vi "Main.vi"() -> ()   [LabVIEW 2026]
uses:
  <vilib>/Instr/_visa.llb/VISA Configure Serial Port (Instr).vi
panel:
  out "Estado de Conexión":string
  in  "RESET SLAVE":bool
  out "maquina":T1(ring)
  out "SR MODO":enum16{"AUTOMATICO", "MANUAL"}(ring)=enum."MANUAL"
  out "Boton Reset":string
  out "Errores CRC":dbl
  out "Tramas OK":dbl
  out "Estados de la Planta":string
  out "SALIDA PWM":dbl(graph)
  in  "MODO":bool=TRUE
  in  "RESET":bool
  in  "EMERGENCIA":bool
  in  "PWM":dbl=10.0 min=0.0 max=100.0
  out "SP Vs ALTURA":cluster{dbl, dbl}(graph)
  out "PING PONG":dbl(slide) scale=0.0..50.0
  out "PID":T2(ring)
  out "error out":errorcluster
  out "Enum":enum16{"DESCONECTADO", "CONECTADO"}(ring)
  out "ESTADO  SYS":enum16{"DETENIDO", "EJECUTANDO", "ERROR"}(ring)
  in  "PARADA":bool
  in  "INICIO":bool
  out "PID":string
  in  "SP":dbl=25.0 min=0.0 max=100.0
  in  "KD":dbl=0.07 min=0.0 max=65535.0
  in  "KI":dbl=0.14 min=0.0 max=65535.0
  in  "KP":dbl=3.9 min=0.0 max=65535.0
  in  "PID":bool
  out "PWM (%)":dbl format="%.2g"
  out "ERROR (CM)":dbl format="%.2g"
  out "ALTURA (CM)":dbl format="%.2g"
  out "SP (CM)":dbl format="%.2f"
  out "array":string[][](array[string])
  out "Procesar":string
  in  "Stop Simulation":bool
  in  "Numeric":u32=115200
  in  "VISA resource name":refnum<visa-resource-name>="COM12"
  out "Iteracion":i32
  # "Sistema Levitador Neumático"
  # "Planta"
  # "Grafico en Tiempo Real"
  # "COMUNICACIÓN"
  # "ESTADO DEL SISTEMA"
  # "Estado :"
  # "Puerto :"
  # "Comunicación :"
  # "Baud :"
  # "Estado PID :"
  # "CONFIGURACIÓN PID"
  # "VARIABLES EN TIEMPO REAL"
  # "KP :"
  # "KI :"
  # "KD :"
  # "AUTO"
  # "MANUAL"
  # "SP :"
  # "PWM :"
  # "Mensaje a Procesar :"
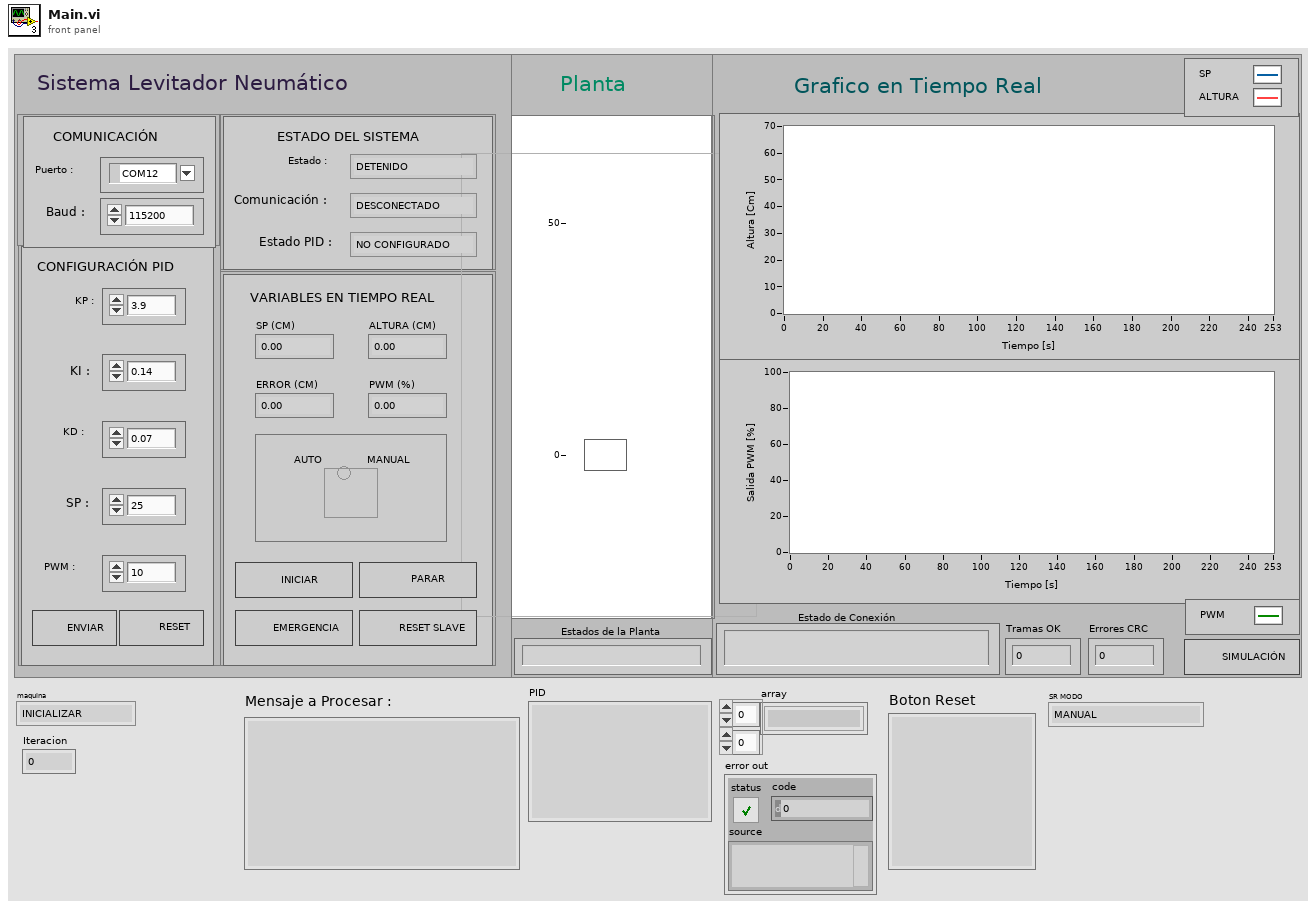
[diagram p1: front panel]
types:
  T1 = enum16{"INICIALIZAR", "ESPERA", "ENVIAR_MODO", "ENVIAR_SP", "ENVIAR_PID", "RECIBIR", "PROCESAR", "ENVIAR_RESET", "ENVIAR_RUN", "ENVIAR_STOP", "ENVIAR_EMERGENCIA_ON", "ENVIAR_EMERGENCIA_OFF", "SLAVE", "ERROR", "CERRAR"}
  T2 = enum16{"NO CONFIGURADO", "CONFIGURADO", "AUTOMATICO"}
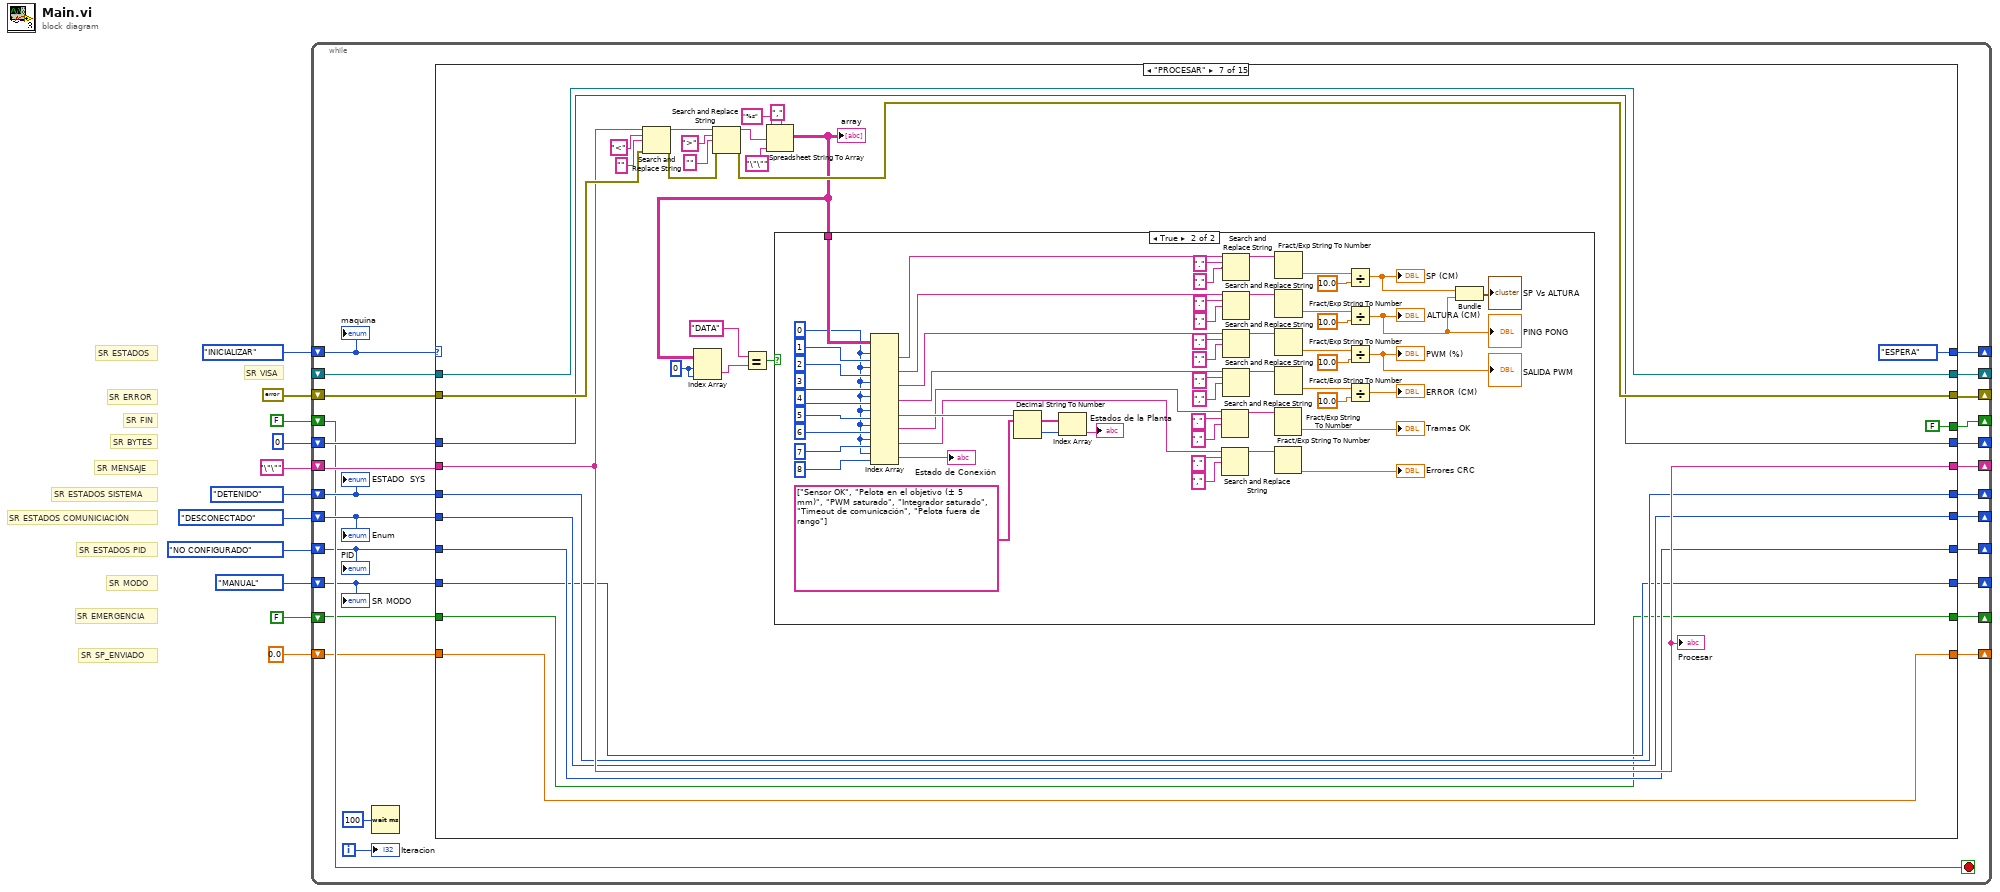
[diagram p0: block diagram]
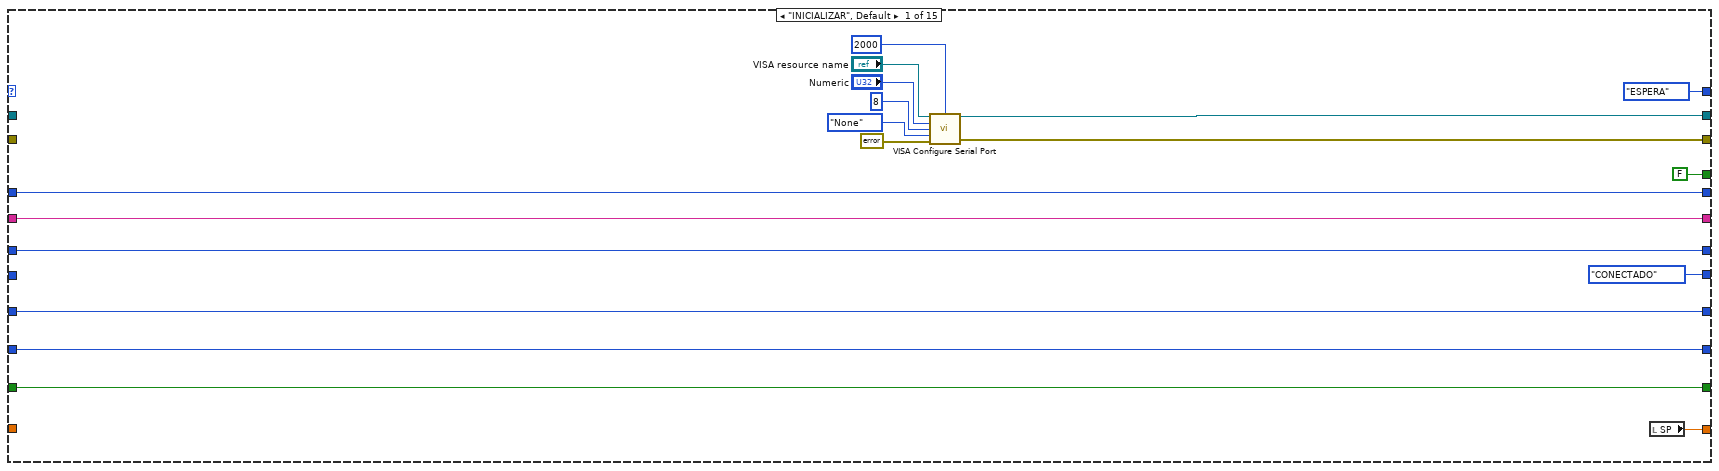
[diagram p2: hidden frame]
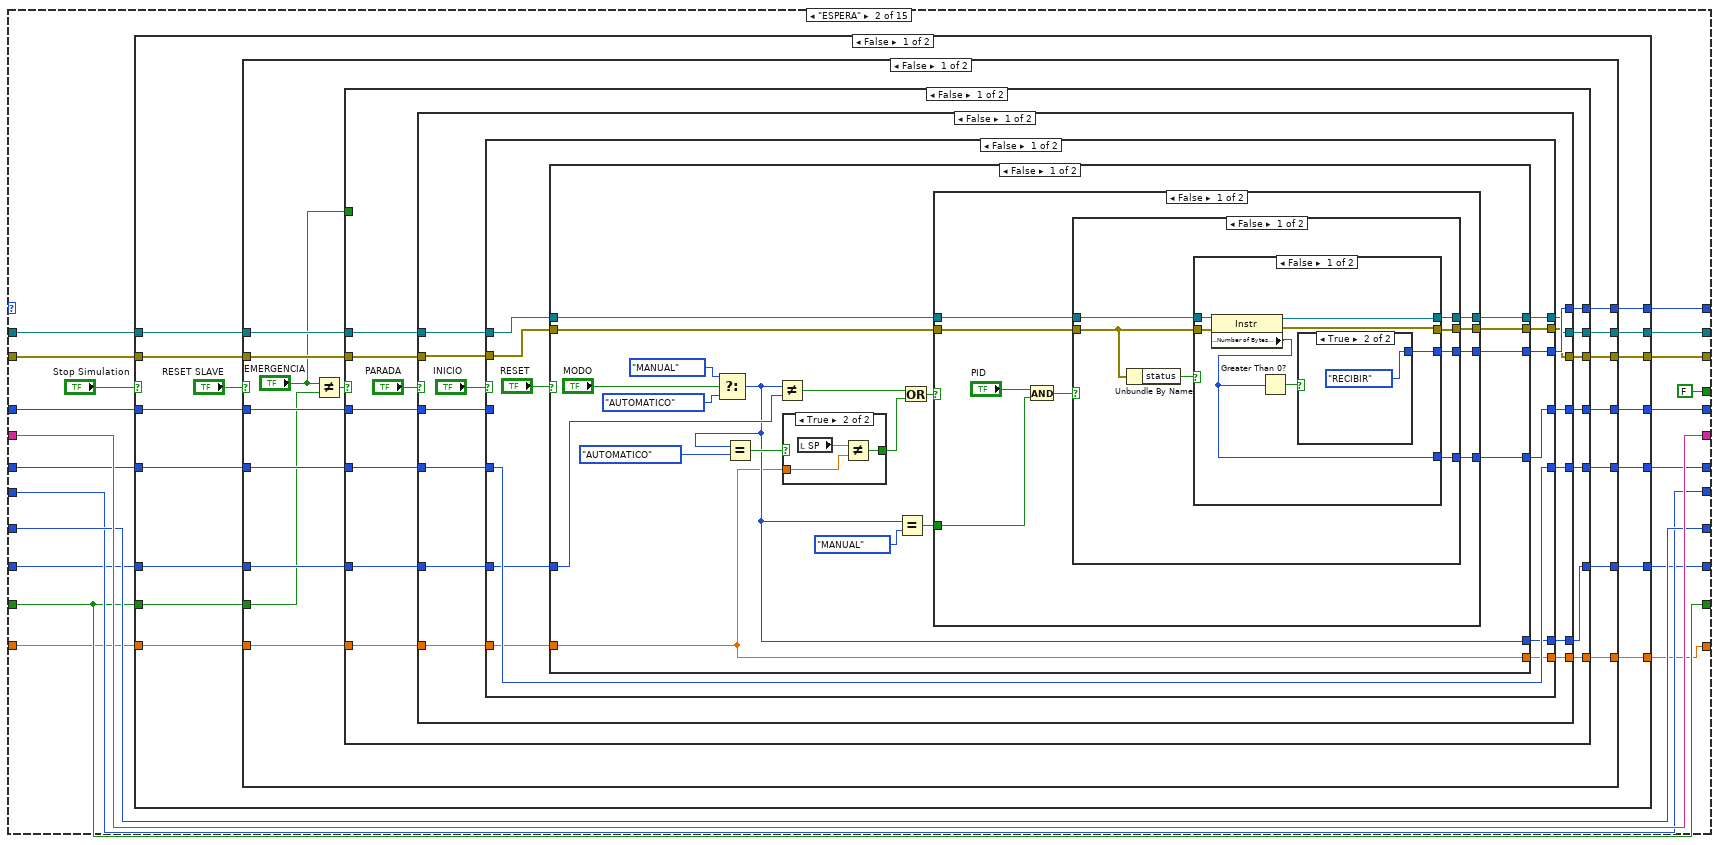
[diagram p3: hidden frame]
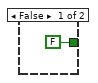
[diagram p4: hidden frame]
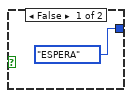
[diagram p5: hidden frame]
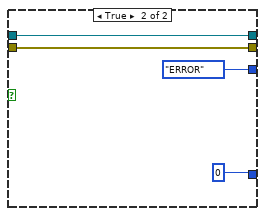
[diagram p6: hidden frame]
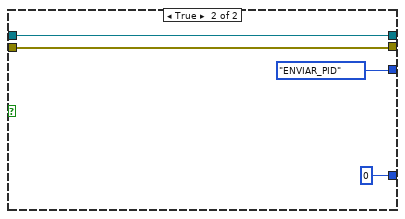
[diagram p7: hidden frame]
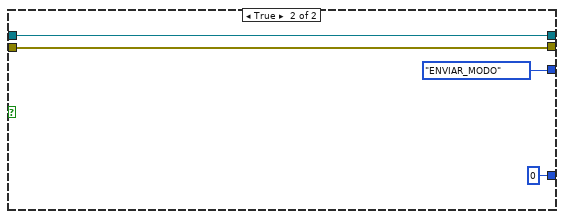
[diagram p8: hidden frame]
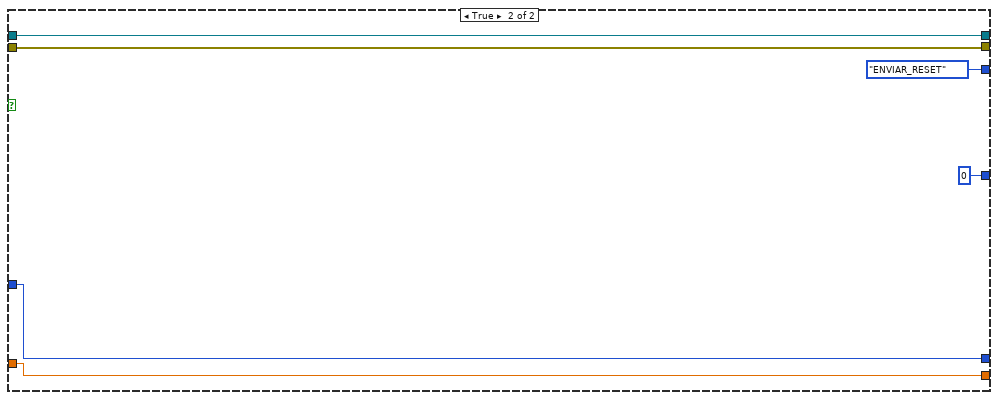
[diagram p9: hidden frame]
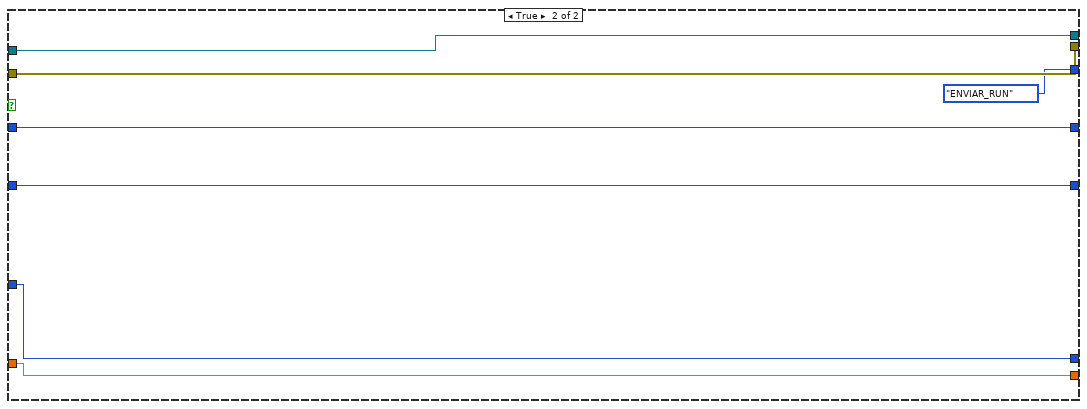
[diagram p10: hidden frame]
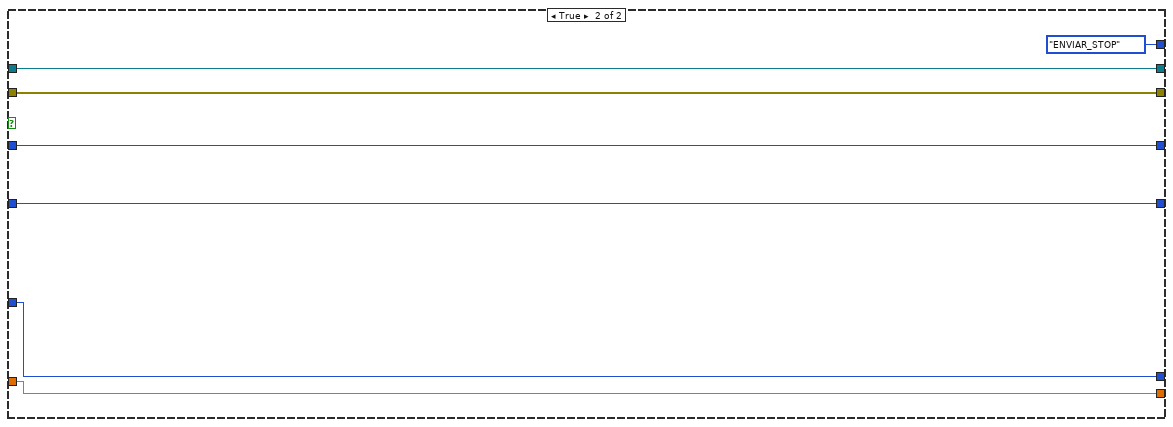
[diagram p11: hidden frame]
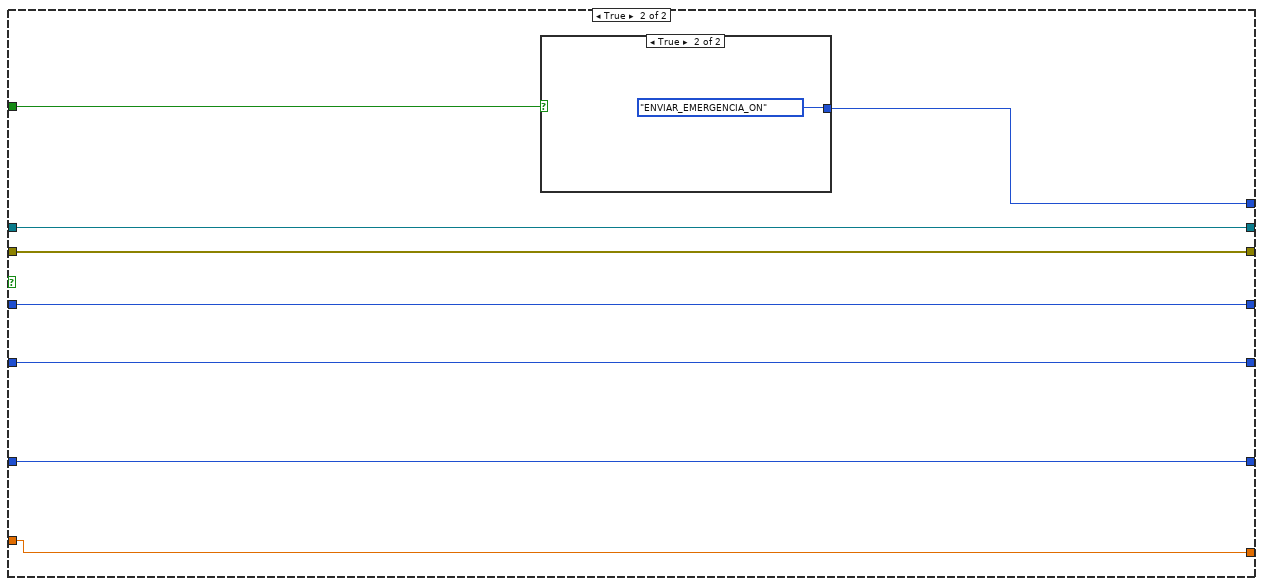
[diagram p12: hidden frame]
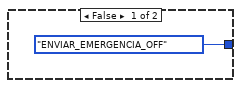
[diagram p13: hidden frame]
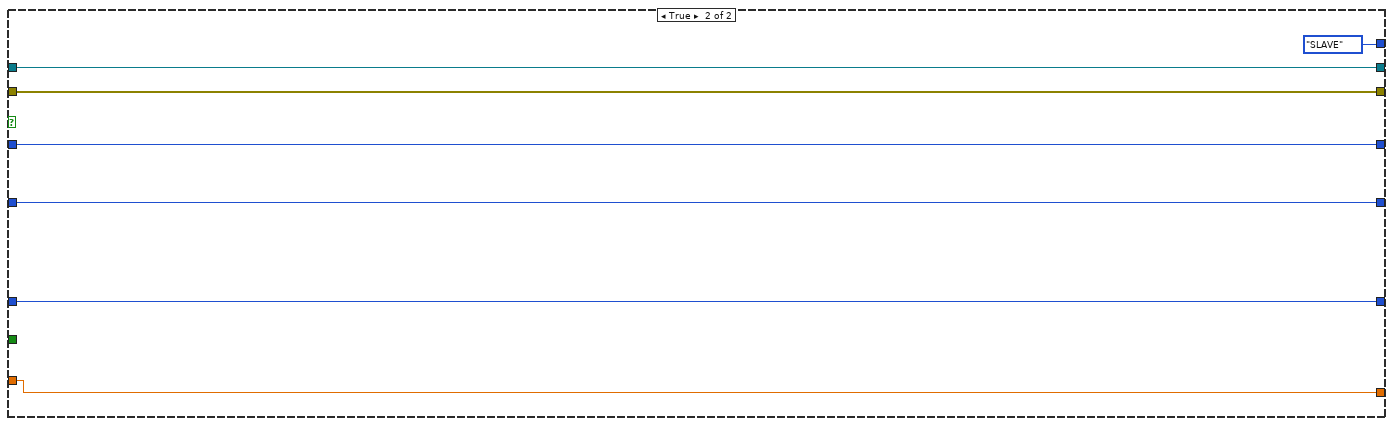
[diagram p14: hidden frame]
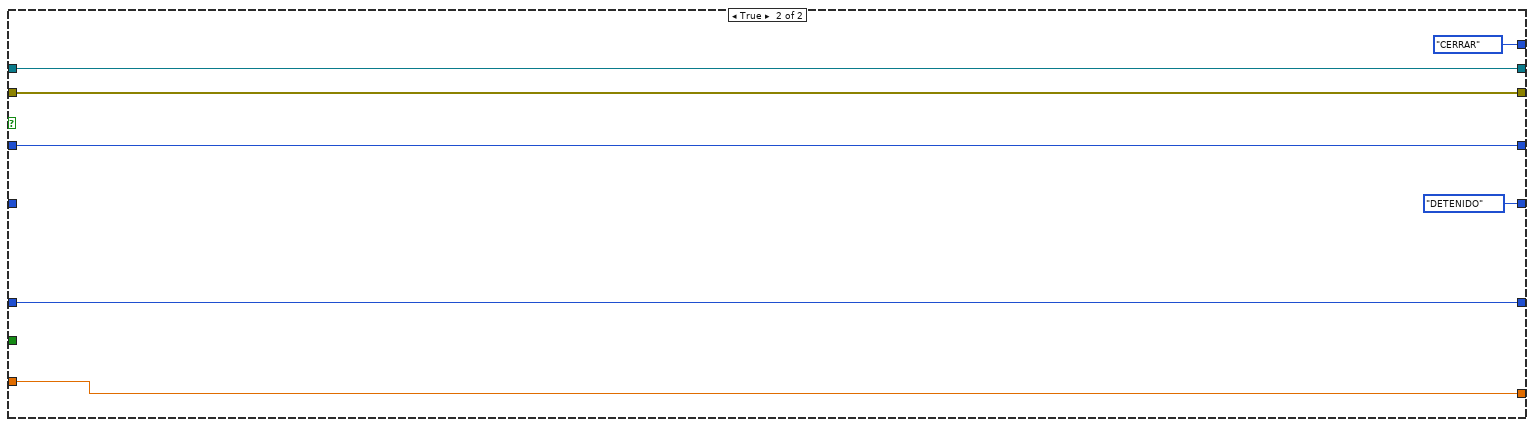
[diagram p15: hidden frame]
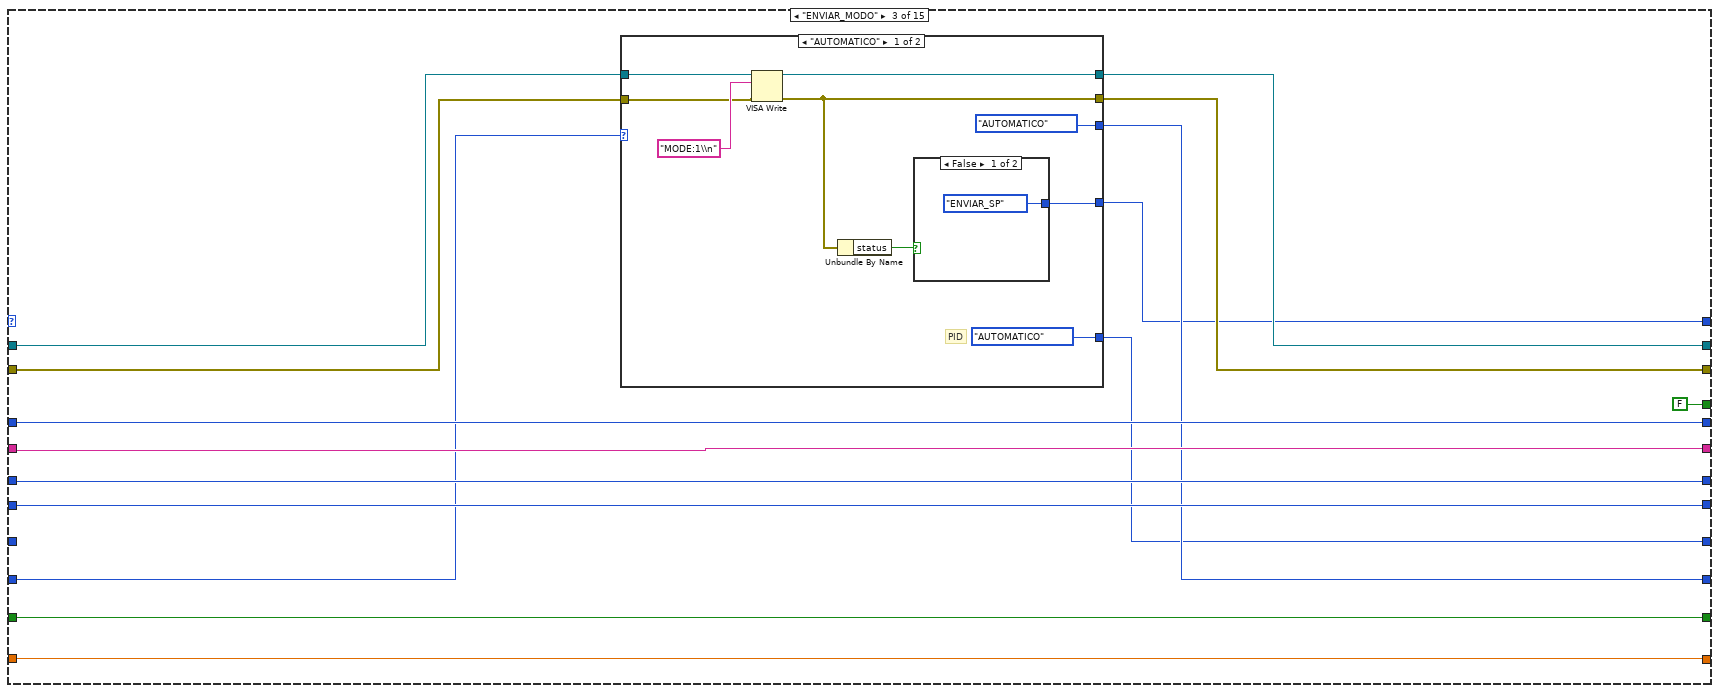
[diagram p16: hidden frame]
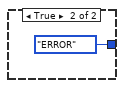
[diagram p17: hidden frame]
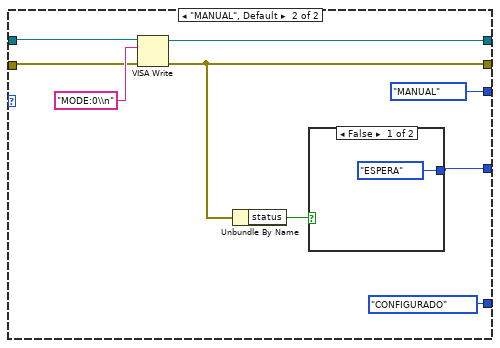
[diagram p18: hidden frame]
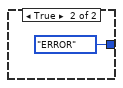
[diagram p19: hidden frame]
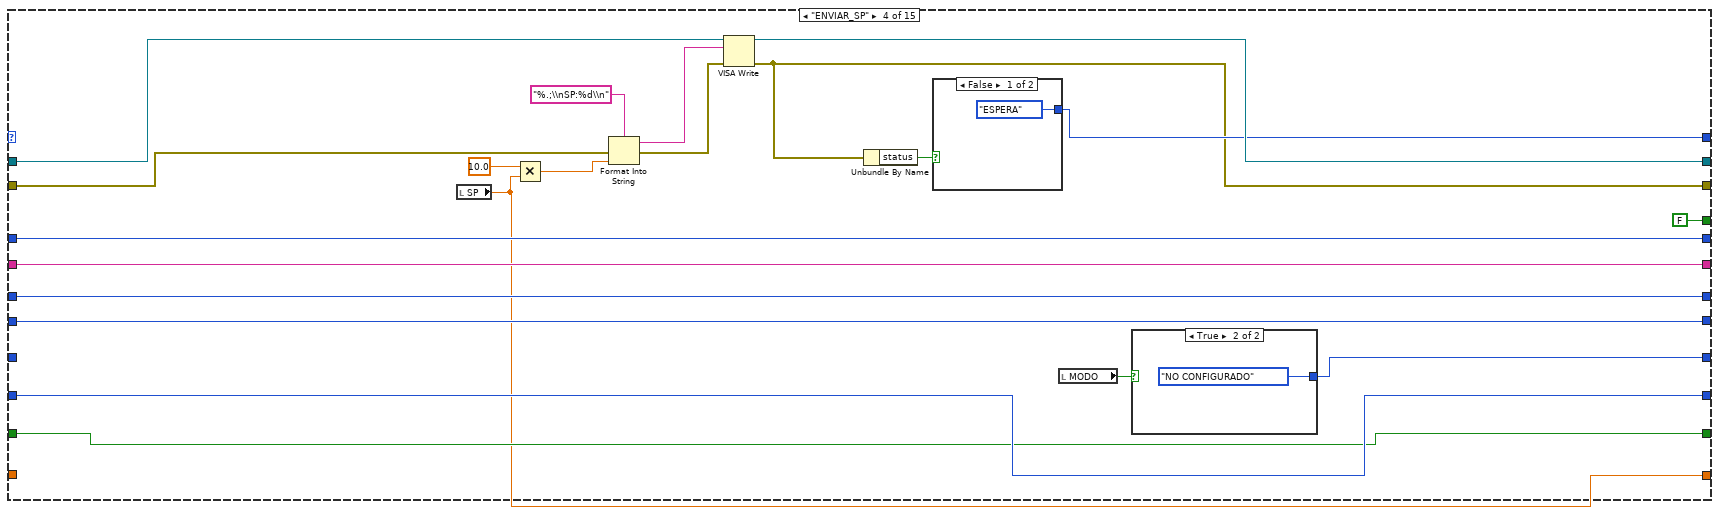
[diagram p20: hidden frame]
diagram:
  # "SR SP_ENVIADO"
  # "SR EMERGENCIA"
  # "SR MODO"
  # "SR ESTADOS PID"
  # "SR ESTADOS COMUNICIACIÓN"
  # "SR ESTADOS SISTEMA"
  # "SR MENSAJE"
  # "SR BYTES"
  # "SR FIN"
  # "SR ERROR"
  # "SR ESTADOS"
  # "SR VISA"
  n1 = while {
    shift-right: [w35] -> _
    shift-left: _ -> [w33]
    shift-right: [w34] -> _
    shift-left: errorcluster {"status"=FALSE, "code"=0, "source"=""} ("error out") -> [w32]
    shift-right: [w31] -> _
    shift-left: FALSE -> [w22]
    shift-right: [w30] -> _
    shift-left: u32 0 ("Bytes at Port") -> [w29]
    shift-right: [w28] -> _
    shift-left: "\"\"" -> [w27]
    shift-right: [w23] -> _
    shift-left: enum16{"DETENIDO", "EJECUTANDO", "ERROR"}."DETENIDO" -> [w25]
    shift-right: [w24] -> _
    shift-left: enum16{"DESCONECTADO", "CONECTADO"}."DESCONECTADO" -> [w26]
    shift-right: [w20] -> _
    shift-left: T2."NO CONFIGURADO" -> [w21]
    shift-right: [w18] -> _
    shift-left: T1."INICIALIZAR" -> [w19]
    shift-right: [w16] -> _
    shift-left: enum16{"AUTOMATICO", "MANUAL"}."MANUAL" -> [w17]
    shift-right: [w14] -> _
    shift-left: FALSE -> [w15]
    shift-right: [w12] -> _
    shift-left: 0.0 -> [w13]
    i -> [w37]
    stop <- w22 stop-if-true
    n2 = Wait (ms)(milliseconds to wait=u32 100) -> ()  [unwired: 1 out]
    n3 = case shown="\"PROCESAR\"" w19 {
      tunnel: [T1."ESPERA" w59 w253 w293 w333 w353 T1."ESPERA" w455 w476 w492 w512 w530 T1."CERRAR" T1."CERRAR" w567] -> w18
      tunnel: [w49 w72 w257 w294 w338 w358 w391 w457 w478 w493 w509 w532 w550 w556 w566] -> w35
      tunnel: [w48 w71 w256 w292 w335 w355 w382 w452 w477 w494 w508 w531 w546 w557 w565] -> w34
      tunnel: w33 -> [_ w73 w259 w296 w339 w360 w391 w459 w480 w498 w514 w534 w550 w556 w569]
      tunnel: w32 -> [_ w67 w258 w295 w341 w359 w383 w458 w479 w497 w513 w533 w546 w558 w568]
      tunnel: [FALSE FALSE FALSE FALSE FALSE FALSE FALSE FALSE FALSE FALSE FALSE FALSE FALSE TRUE FALSE] -> w31
      tunnel: [w46 w70 w262 w304 w343 w357 w378 w448 w473 w495 w510 w527 w548 w562 w570] -> w30
      tunnel: w29 -> [w46 w69 w262 w304 w343 w357 w378 w448 w473 w495 w510 w527 w548 w562 w570]
      tunnel: [w45 w68 w263 w305 w342 w356 w376 w454 w474 w496 w507 w526 w547 w561 w571] -> w28
      tunnel: w27 -> [w45 w68 w263 w305 w342 _ w376 w454 w474 w496 w507 w526 w547 w561 w571]
      tunnel: w25 -> [w44 w65 w261 w307 w332 w352 w370 w453 _ _ _ w523 w545 _ w572]
      tunnel: w26 -> [_ w62 w260 w303 w316 w350 w368 w451 w470 w488 w506 w524 w543 _ w573]
      tunnel: [enum16{"DESCONECTADO", "CONECTADO"}."CONECTADO" w62 w260 w303 w316 w350 w368 w451 w470 w488 w506 w524 w543 enum16{"DESCONECTADO", "CONECTADO"}."DESCONECTADO" w573] -> w24
      tunnel: [w44 w66 w261 w307 w332 w352 w370 w453 enum16{"DETENIDO", "EJECUTANDO", "ERROR"}."EJECUTANDO" enum16{"DETENIDO", "EJECUTANDO", "ERROR"}."DETENIDO" enum16{"DETENIDO", "EJECUTANDO", "ERROR"}."DETENIDO" w523 w545 enum16{"DETENIDO", "EJECUTANDO", "ERROR"}."DETENIDO" w572] -> w23
      tunnel: w21 -> [w43 w63 _ _ _ w351 w369 _ w471 w489 w511 w528 w544 w555 w574]
      tunnel: [w43 w63 w252 w291 T2."CONFIGURADO" w351 w369 T2."NO CONFIGURADO" w471 w489 w511 w528 w544 w555 w574] -> w20
      tunnel: w17 -> [w41 w61 w254 w289 w314 w349 w367 w449 w469 w487 w505 w525 w542 w554 w575]
      tunnel: [w41 w60 w255 w289 w314 w349 w367 w449 w469 w487 w505 w525 w542 w554 w575] -> w16
      tunnel: w15 -> [w40 w58 w251 w288 w313 w348 w366 w447 w468 w486 _ _ w541 w553 _]
      tunnel: [w40 w58 w251 w288 w313 w348 w366 w447 w468 w486 TRUE FALSE w541 w553 FALSE] -> w14
      tunnel: w13 -> [_ w57 w250 _ w312 w347 w365 w446 w467 w485 w503 w521 w540 w552 w576]
      tunnel: [w39 w56 w250 w287 w312 w347 w365 w446 w467 w485 w503 w521 w540 w552 w576] -> w12
      frame "INICIALIZAR", Default {
        n4 = call-poly "VISA Configure Serial Port"("VISA resource name"="VISA resource name", "timeout (10sec)"=u32 2000, "baud rate (9600)"="Numeric", "data bits (8)"=u16 8, "parity (0:none)"=enum16{"None", "Odd", "Even", "Mark", "Space"}."None", "error in (no error)"=errorcluster {"status"=FALSE, "code"=0, "source"=""}) -> ("VISA resource name out"=w49:refnum<visa-resource-name>, "error out"=w48:errorcluster)  [unwired: 8 in]
        n5 = local read "SP"() -> (w39:dbl)
      }
      frame "ESPERA" {
        n6 = case shown="False" "Stop Simulation" {
          tunnel: [w89 T1."CERRAR"] -> w59
          tunnel: w73 -> [w88 w247]
          tunnel: [w87 w247] -> w72
          tunnel: [w86 w246] -> w71
          tunnel: [w85 w249] -> w70
          tunnel: w69 -> [w84 w249]
          tunnel: w67 -> [w83 w246]
          tunnel: [w82 enum16{"DETENIDO", "EJECUTANDO", "ERROR"}."DETENIDO"] -> w66
          tunnel: w65 -> [w81 _]
          tunnel: w61 -> [w80 w245]
          tunnel: [w79 w245] -> w60
          tunnel: w58 -> [w78 _]
          tunnel: w57 -> [w77 w244]
          tunnel: [w76 w244] -> w56
          frame False {
            n7 = case shown="False" "RESET SLAVE" {
              tunnel: [w105 T1."SLAVE"] -> w89
              tunnel: w88 -> [w104 w237]
              tunnel: [w103 w237] -> w87
              tunnel: [w102 w238] -> w86
              tunnel: [w101 w239] -> w85
              tunnel: w84 -> [w100 w239]
              tunnel: w83 -> [w99 w238]
              tunnel: [w98 w240] -> w82
              tunnel: w81 -> [w97 w240]
              tunnel: w80 -> [w96 w241]
              tunnel: [w95 w241] -> w79
              tunnel: w78 -> [w93 _]
              tunnel: w77 -> [w91 w242]
              tunnel: [w90 w242] -> w76
              frame False {
                n8 = Not Equal?(x="EMERGENCIA", y=w93) -> (x != y?=w94:bool)
                n9 = case shown="False" w94 {
                  tunnel: [w119 w228] -> w105
                  tunnel: w104 -> [w111 w231]
                  tunnel: [w118 w231] -> w103
                  tunnel: [w117 w230] -> w102
                  tunnel: [w116 w233] -> w101
                  tunnel: w100 -> [w115 w233]
                  tunnel: w99 -> [w110 w230]
                  tunnel: [w113 w232] -> w98
                  tunnel: w97 -> [w112 w232]
                  tunnel: w96 -> [w109 w229]
                  tunnel: [w108 w229] -> w95
                  tunnel: "EMERGENCIA" -> [_ w227]
                  tunnel: w91 -> [w107 w226]
                  tunnel: [w106 w226] -> w90
                  frame False {
                    n10 = case shown="False" "PARADA" {
                      tunnel: [w133 T1."ENVIAR_STOP"] -> w119
                      tunnel: w111 -> [w132 w225]
                      tunnel: w110 -> [w131 w224]
                      tunnel: [w130 w225] -> w118
                      tunnel: [w129 w224] -> w117
                      tunnel: [w128 w223] -> w116
                      tunnel: w115 -> [w126 w223]
                      tunnel: [w125 w222] -> w113
                      tunnel: w112 -> [w124 w222]
                      tunnel: w109 -> [w123 w221]
                      tunnel: [w122 w221] -> w108
                      tunnel: w107 -> [w121 w220]
                      tunnel: [w120 w220] -> w106
                      frame False {
                        n11 = case shown="False" "INICIO" {
                          tunnel: [w145 T1."ENVIAR_RUN"] -> w133
                          tunnel: w132 -> [w144 w218]
                          tunnel: w131 -> [w143 w217]
                          tunnel: [w142 w218] -> w130
                          tunnel: [w141 w217] -> w129
                          tunnel: [w140 w216] -> w128
                          tunnel: w126 -> [_ w216]
                          tunnel: [w139 w215] -> w125
                          tunnel: w124 -> [w139 w215]
                          tunnel: w123 -> [w137 w214]
                          tunnel: [w136 w214] -> w122
                          tunnel: w121 -> [w135 w213]
                          tunnel: [w134 w213] -> w120
                          frame False {
                            n12 = case shown="False" "RESET" {
                              tunnel: [w164 T1."ENVIAR_RESET"] -> w145
                              tunnel: w144 -> [w163 w211]
                              tunnel: w143 -> [w162 w210]
                              tunnel: [w161 w211] -> w142
                              tunnel: [w160 w210] -> w141
                              tunnel: [w159 u32 0 ("Bytes at Port")] -> w140
                              tunnel: w137 -> [w155 w208]
                              tunnel: [w148 w208] -> w136
                              tunnel: w135 -> [w146 w207]
                              tunnel: [w146 w207] -> w134
                              frame False {
                                n13 = Select(t=enum16{"AUTOMATICO", "MANUAL"}."MANUAL", s="MODO", f=enum16{"AUTOMATICO", "MANUAL"}."AUTOMATICO") -> (s? t:f=w148:enum16{"AUTOMATICO", "MANUAL"})
                                n14 = Equal?(x=w148, y=enum16{"AUTOMATICO", "MANUAL"}."AUTOMATICO") -> (x = y?=w149:bool)
                                n15 = Not Equal?(x=w148, y=w155) -> (x != y?=w151:bool)
                                n16 = case shown="True" w149 {
                                tunnel: [FALSE w167] -> w152
                                tunnel: w146 -> [_ w166]
                                frame False {
                                }
                                frame True {
                                n17 = local read "SP"() -> (w168:dbl)
                                n18 = Not Equal?(x=w168, y=w166) -> (x != y?=w167:bool)
                                }
                                }
                                n19 = Equal?(x=w148, y=enum16{"AUTOMATICO", "MANUAL"}."MANUAL") -> (x = y?=w154:bool)
                                n20 = Or(x=w151, y=w152) -> (x .or. y?=w150:bool)
                                n21 = case shown="False" w150 {
                                tunnel: [w177 T1."ENVIAR_MODO"] -> w164
                                tunnel: w163 -> [w176 w205]
                                tunnel: w162 -> [w175 w204]
                                tunnel: [w174 w205] -> w161
                                tunnel: [w173 w204] -> w160
                                tunnel: [w172 u32 0 ("Bytes at Port")] -> w159
                                tunnel: w154 -> [w171 _]
                                frame False {
                                n22 = And(x="PID", y=w171) -> (x .and. y?=w169:bool)
                                n23 = case shown="False" w169 {
                                tunnel: [w184 T1."ENVIAR_PID"] -> w177
                                tunnel: w176 -> [w183 w200]
                                tunnel: w175 -> [w179 w199]
                                tunnel: [w182 w200] -> w174
                                tunnel: [w181 w199] -> w173
                                tunnel: [w180 u32 0 ("Bytes at Port")] -> w172
                                frame False {
                                n24 = Unbundle By Name(w179) -> ("status"=w178:bool)
                                n25 = case shown="False" w178 {
                                tunnel: [w191 T1."ERROR"] -> w184
                                tunnel: w183 -> [w190 w197]
                                tunnel: w179 -> [w189 w196]
                                tunnel: [w188 w197] -> w182
                                tunnel: [w187 w196] -> w181
                                tunnel: [w185 u32 0 ("Bytes at Port")] -> w180
                                frame False {
                                n26 = property class="Instr"(reference=w190, error in=w189) -> (reference out=w188:refnum<visa-resource-name>, error out=w187:errorcluster, "Serial Settings:Number of Bytes at Serial Port"=w185:u32)
                                n27 = Greater Than 0?(x=w185) -> (x > 0?=w186:bool)
                                n28 = case shown="True" w186 {
                                tunnel: [T1."ESPERA" T1."RECIBIR"] -> w191
                                frame False {
                                }
                                frame True {
                                }
                                }
                                }
                                frame True {
                                }
                                }
                                }
                                frame True {
                                }
                                }
                                }
                                frame True {
                                }
                                }
                              }
                              frame True {
                              }
                            }
                          }
                          frame True {
                          }
                        }
                      }
                      frame True {
                      }
                    }
                  }
                  frame True {
                    n29 = case shown="True" w227 {
                      tunnel: [T1."ENVIAR_EMERGENCIA_OFF" T1."ENVIAR_EMERGENCIA_ON"] -> w228
                      frame False {
                      }
                      frame True {
                      }
                    }
                  }
                }
              }
              frame True {
              }
            }
          }
          frame True {
          }
        }
      }
      frame "ENVIAR_MODO" {
        n30 = case shown="\"AUTOMATICO\"" w254 {
          tunnel: w259 -> [w271 w283]
          tunnel: w258 -> [w270 w282]
          tunnel: [w269 w280] -> w257
          tunnel: [w268 w281] -> w256
          tunnel: [enum16{"AUTOMATICO", "MANUAL"}."AUTOMATICO" enum16{"AUTOMATICO", "MANUAL"}."MANUAL"] -> w255
          tunnel: [w266 w277] -> w253
          tunnel: [T2."AUTOMATICO" T2."CONFIGURADO"] -> w252
          frame "AUTOMATICO" {
            # "PID"
            n31 = VISA Write(VISA resource name=w271, write buffer="MODE:1\\n", error in (no error)=w270) -> (VISA resource name out=w269:refnum<visa-resource-name>, error out=w268:errorcluster)  [unwired: 1 out]
            n32 = Unbundle By Name(w268) -> ("status"=w272:bool)
            n33 = case shown="False" w272 {
              tunnel: [T1."ENVIAR_SP" T1."ERROR"] -> w266
              frame False {
              }
              frame True {
              }
            }
          }
          frame "MANUAL", Default {
            n34 = VISA Write(VISA resource name=w283, write buffer="MODE:0\\n", error in (no error)=w282) -> (VISA resource name out=w280:refnum<visa-resource-name>, error out=w281:errorcluster)  [unwired: 1 out]
            n35 = Unbundle By Name(w281) -> ("status"=w279:bool)
            n36 = case shown="False" w279 {
              tunnel: [T1."ESPERA" T1."ERROR"] -> w277
              frame False {
              }
              frame True {
              }
            }
          }
        }
      }
      frame "ENVIAR_SP" {
        n37 = local read "SP"() -> (w287:dbl)
        n38 = Multiply(x=10.0, y=w287) -> (x*y=w300:dbl)
        n39 = Format Into String(format string="%.;\\nSP:%d\\n", error in=w295, w300) -> (resulting string=w302:string, error out=w301:errorcluster)  [unwired: 1 in]
        n40 = VISA Write(VISA resource name=w296, write buffer=w302, error in (no error)=w301) -> (VISA resource name out=w294:refnum<visa-resource-name>, error out=w292:errorcluster)  [unwired: 1 out]
        n41 = Unbundle By Name(w292) -> ("status"=w299:bool)
        n42 = case shown="False" w299 {
          tunnel: [T1."ESPERA" T1."ERROR"] -> w293
          frame False {
          }
          frame True {
          }
        }
        n43 = local read "MODO"() -> (w290:bool)
        n44 = case shown="True" w290 {
          tunnel: [T2."AUTOMATICO" T2."NO CONFIGURADO"] -> w291
          frame False {
          }
          frame True {
          }
        }
      }
      frame "ENVIAR_PID" {
        n45 = Multiply(x=100.0, y="KP") -> (x*y=w323:dbl)
        n46 = Multiply(x=100.0, y="KI") -> (x*y=w327:dbl)
        n47 = Multiply(x=100.0, y="KD") -> (x*y=w331:dbl)
        n48 = Multiply(x=10.0, y="SP") -> (x*y=w320:dbl)
        n49 = Multiply(x=10.0, y="PWM") -> (x*y=w317:dbl)
        n50 = Format Into String(format string="%.;\\nKP:%d\\nKI:%d\\nKD:%d\\nSP:%d\\nPWM:%d\\n", error in=w341, w323, w327, w331, w320, w317) -> (resulting string=w340:string, error out=w336:errorcluster)  [unwired: 1 in]
        "PID" <- w340
        n51 = VISA Write(VISA resource name=w339, write buffer=w340, error in (no error)=w336) -> (VISA resource name out=w338:refnum<visa-resource-name>, error out=w335:errorcluster)  [unwired: 1 out]
        n52 = Unbundle By Name(w335) -> ("status"=w334:bool)
        n53 = case shown="False" w334 {
          tunnel: [T1."ESPERA" T1."ERROR"] -> w333
          frame False {
          }
          frame True {
          }
        }
      }
      frame "RECIBIR" {
        n54 = VISA Read(VISA resource name=w360, byte count=w357, error in (no error)=w359) -> (VISA resource name out=w358:refnum<visa-resource-name>, read buffer=w356:string, error out=w355:errorcluster)  [unwired: 1 out]
        n55 = Unbundle By Name(w355) -> ("status"=w354:bool)
        n56 = case shown="False" w354 {
          tunnel: [T1."PROCESAR" T1."ERROR"] -> w353
          frame False {
          }
          frame True {
          }
        }
      }
      frame "PROCESAR" {
        w375 = 0 ("index (row)")
        n57 = Search and Replace String(input string=w376, search string="<", replace string="" ("replace string (\"\")"), error in=w383) -> (result string=w387:string, error out=w386:errorcluster)  [unwired: 4 in, 2 out]
        n58 = Search and Replace String(input string=w387, search string=">", replace string="" ("replace string (\"\")"), error in=w386) -> (result string=w380:string, error out=w382:errorcluster)  [unwired: 4 in, 2 out]
        n59 = Spreadsheet String To Array(delimiter (Tab)=",", format string="%s", spreadsheet string=w380, array type (2D Dbl)="\"\"") -> (array=w371:string[][])
        "array" <- w371
        n60 = Index Array(array=w371, index (row)=w375, index (col)=w375) -> (element=w374:string)
        n61 = Equal?(x="DATA", y=w374) -> (x = y?=w372:bool)
        n62 = case shown="True" w372 {
          tunnel: w371 -> [_ w424]
          frame False {
          }
          frame True {
            w394 = 0 ("index (row)")
            n63 = Index Array(array=w424, index (row) #1=w394, index (col) #1=1 ("index"), index (row) #2=w394, index (col) #2=2 ("index"), index (row) #3=w394, index (col) #3=3 ("index"), index (row) #4=w394, index (col) #4=4 ("index"), index (row) #5=w394, index (col) #5=5 ("disabled index (col)"), index (row) #6=w394, index (col) #6=6 ("disabled index (col)"), index (row) #7=w394, index (col) #7=7 ("disabled index (col)"), index (row) #8=w394, index (col) #8=8 ("disabled index (col)")) -> (element #1=w441:string, element #2=w432:string, element #3=w431:string, element #4=w430:string, element #5=w420:string, element #6=w408:string, element #7=w407:string, element #8=→"Estado de Conexión":string)
            n64 = Decimal String To Number(string=w420) -> (number=w418:i32)  [unwired: 2 in, 1 out]
            n65 = Index Array(array=string[] ["Sensor OK", "Pelota en el objetivo (± 5 mm)", "PWM saturado", "Integrador saturado", "Timeout de comunicación", "Pelota fuera de rango"], index=w418) -> (element=→"Estados de la Planta":string)
            n66 = Search and Replace String(input string=w408, search string=".", replace string="," ("replace string (\"\")")) -> (result string=w410:string)  [unwired: 5 in, 3 out]
            n67 = Search and Replace String(input string=w407, search string=".", replace string="," ("replace string (\"\")")) -> (result string=w409:string)  [unwired: 5 in, 3 out]
            n68 = Search and Replace String(input string=w441, search string=".", replace string="," ("replace string (\"\")")) -> (result string=w439:string)  [unwired: 5 in, 3 out]
            n69 = Search and Replace String(input string=w432, search string=".", replace string="," ("replace string (\"\")")) -> (result string=w428:string)  [unwired: 5 in, 3 out]
            n70 = Search and Replace String(input string=w431, search string=".", replace string="," ("replace string (\"\")")) -> (result string=w427:string)  [unwired: 5 in, 3 out]
            n71 = Search and Replace String(input string=w430, search string=".", replace string="," ("replace string (\"\")")) -> (result string=w426:string)  [unwired: 5 in, 3 out]
            n72 = Fract/Exp String To Number(string=w410) -> (number=→"Tramas OK":dbl)  [unwired: 3 in, 1 out]
            n73 = Fract/Exp String To Number(string=w409) -> (number=→"Errores CRC":dbl)  [unwired: 3 in, 1 out]
            n74 = Fract/Exp String To Number(string=w439) -> (number=w422:dbl)  [unwired: 3 in, 1 out]
            n75 = Fract/Exp String To Number(string=w428) -> (number=w402:dbl)  [unwired: 3 in, 1 out]
            n76 = Fract/Exp String To Number(string=w427) -> (number=w399:dbl)  [unwired: 3 in, 1 out]
            n77 = Fract/Exp String To Number(string=w426) -> (number=w396:dbl)  [unwired: 3 in, 1 out]
            n78 = Divide(x=w422, y=10.0) -> (x/y=w404:dbl)
            "SP (CM)" <- w404
            n79 = Divide(x=w402, y=10.0) -> (x/y=w401:dbl)
            "ALTURA (CM)" <- w401
            "PING PONG" <- w401
            n80 = Divide(x=w399, y=10.0) -> (x/y=→"PWM (%)" →"SALIDA PWM":dbl)
            n81 = Divide(x=w396, y=10.0) -> (x/y=→"ERROR (CM)":dbl)
            n82 = Bundle(w404, w401) -> (→"SP Vs ALTURA":cluster{dbl, dbl})  [unwired: 1 in]
          }
        }
        "Procesar" <- w376
      }
      frame "ENVIAR_RESET" {
        w460 = 0.0 ("input 1")
        n83 = Format Into String(format string="%.;\\nKP:%d\\nKI:%d\\nKD:%d\\nSP:%d\\nPWM:%d\\n", error in=w458, w460, w460, w460, w460, w460) -> (resulting string=w464:string, error out=w462:errorcluster)  [unwired: 1 in]
        "Boton Reset" <- w464
        n84 = VISA Write(VISA resource name=w459, write buffer=w464, error in (no error)=w462) -> (VISA resource name out=w457:refnum<visa-resource-name>, error out=w452:errorcluster)  [unwired: 1 out]
        n85 = Unbundle By Name(w452) -> ("status"=w461:bool)
        n86 = case shown="False" w461 {
          tunnel: [T1."ESPERA" T1."ERROR"] -> w455
          frame False {
          }
          frame True {
          }
        }
      }
      frame "ENVIAR_RUN" {
        n87 = VISA Write(VISA resource name=w480, write buffer="EN:1\\n", error in (no error)=w479) -> (VISA resource name out=w478:refnum<visa-resource-name>, error out=w477:errorcluster)  [unwired: 1 out]
        n88 = Unbundle By Name(w477) -> ("status"=w482:bool)
        n89 = case shown="False" w482 {
          tunnel: [T1."ESPERA" T1."ERROR"] -> w476
          frame False {
          }
          frame True {
          }
        }
      }
      frame "ENVIAR_STOP" {
        n90 = VISA Write(VISA resource name=w498, write buffer="EN:0\\n", error in (no error)=w497) -> (VISA resource name out=w493:refnum<visa-resource-name>, error out=w494:errorcluster)  [unwired: 1 out]
        n91 = Unbundle By Name(w494) -> ("status"=w500:bool)
        n92 = case shown="False" w500 {
          tunnel: [T1."ESPERA" T1."ERROR"] -> w492
          frame False {
          }
          frame True {
          }
        }
      }
      frame "ENVIAR_EMERGENCIA_ON" {
        n93 = VISA Write(VISA resource name=w514, write buffer="EMG:1\\n", error in (no error)=w513) -> (VISA resource name out=w509:refnum<visa-resource-name>, error out=w508:errorcluster)  [unwired: 1 out]
        n94 = Unbundle By Name(w508) -> ("status"=w518:bool)
        n95 = case shown="False" w518 {
          tunnel: [T1."RECIBIR" T1."ERROR"] -> w512
          frame False {
          }
          frame True {
          }
        }
      }
      frame "ENVIAR_EMERGENCIA_OFF" {
        n96 = VISA Write(VISA resource name=w534, write buffer="EMG:0\\n", error in (no error)=w533) -> (VISA resource name out=w532:refnum<visa-resource-name>, error out=w531:errorcluster)  [unwired: 1 out]
        n97 = Unbundle By Name(w531) -> ("status"=w536:bool)
        n98 = case shown="False" w536 {
          tunnel: [T1."ESPERA" T1."ERROR"] -> w530
          frame False {
          }
          frame True {
          }
        }
      }
      frame "ERROR" {
        "error out" <- w546
      }
      frame "CERRAR" {
        n99 = VISA Close(VISA resource name=w556, error in (no error)=w558) -> (error out=w557:errorcluster)
      }
      frame "SLAVE" {
        n100 = VISA Write(VISA resource name=w569, write buffer="RST:1\\n", error in (no error)=w568) -> (VISA resource name out=w566:refnum<visa-resource-name>, error out=w565:errorcluster)  [unwired: 1 out]
        n101 = Unbundle By Name(w565) -> ("status"=w564:bool)
        n102 = case shown="False" w564 {
          tunnel: [T1."ESPERA" T1."ERROR"] -> w567
          frame False {
          }
          frame True {
          }
        }
      }
    }
    "Iteracion" <- w37
    "ESTADO  SYS" <- w25
    "Enum" <- w26
    "PID" <- w21
    "SR MODO" <- w17
    "maquina" <- w19
  }
